vi "Download Package.vi"(7 "version (latest)":string, 8 "error in":errorcluster, 9 "download all dependencies? (T)":bool=TRUE, 10 "destination folder":path, 11 "package name":string) -> (0 "error out":errorcluster)   [LabVIEW 2014, in "NIPM_API.lvlib"]
doc: "Downloads the package and all its dependencies from registered feeds to a destination folder.\n\nINPUT(s)\n<B>Package name</B>: Specifies the package name of the package you want to download. The package must be in one of your registered feeds.\n\n<B>Destination folder</B>: Specifies the folder to place the downloaded package file(s).\n\n<B>Version (latest)</B>: Specifies the version of the package you want to download. If this input is left unwired, this VI will download the latest version of the package in your registered feeds by default.\n\n<B>Download all dependencies</B>: If you set this to TRUE, this VI will download both the specified package and all of its dependencies."
uses:
  NIPM_API.lvlib
panel:
  out "cmd standard output":string
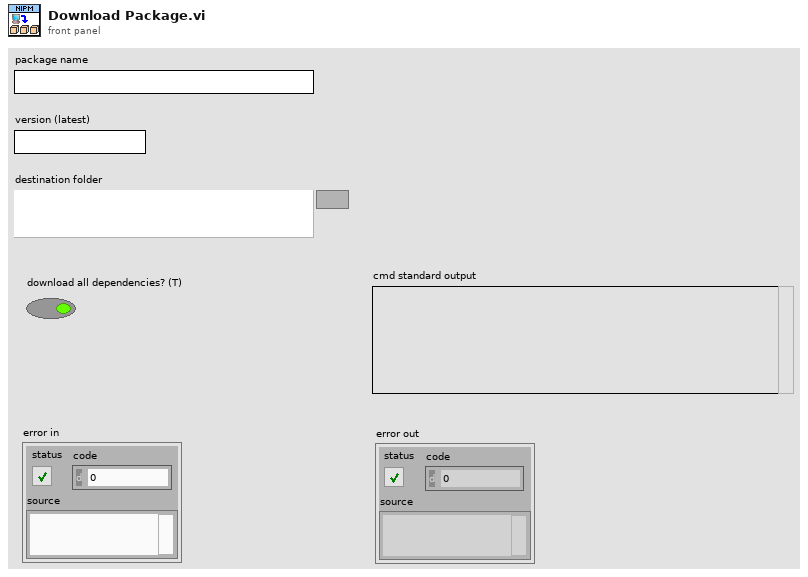
[diagram p1: front panel]
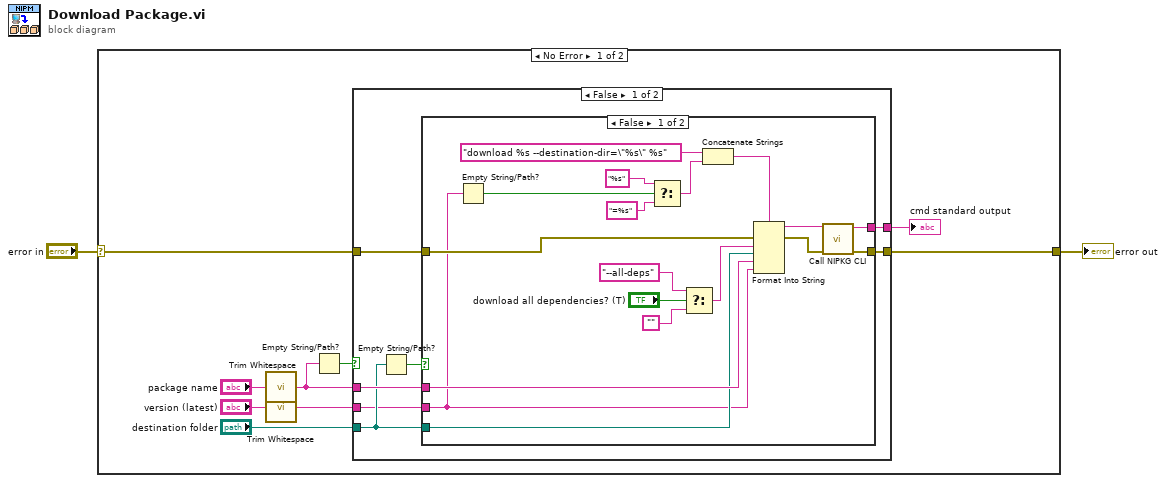
[diagram p0: block diagram]
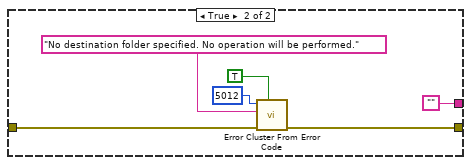
[diagram p2: hidden frame]
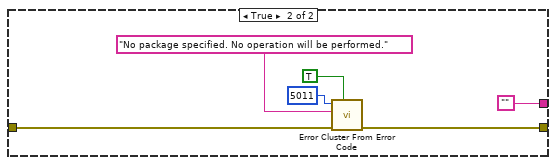
[diagram p3: hidden frame]
diagram:
  n1 = case shown="No Error" "error in" {
    selector: "error in" -> [w11 w49]
    tunnel: [w7 w49] -> w1
    frame No Error {
      n2 = call <vilib>:"Trim Whitespace.vi"("string"="package name") -> ("trimmed string"=w6:string)  [unwired: 1 in]
      n3 = call <vilib>:"Trim Whitespace.vi"("string"="version (latest)") -> ("trimmed string"=w3:string)  [unwired: 1 in]
      n4 = Empty String/Path?(string/path=w6) -> (empty?=w8:bool)
      n5 = case shown="False" w8 {
        tunnel: w11 -> [w18 w44]
        tunnel: "destination folder" -> [w14 _]
        tunnel: w6 -> [w17 _]
        tunnel: [w16 w45] -> w7
        tunnel: [w15 ""] -> w5
        tunnel: w3 -> [w12 _]
        frame False {
          n6 = Empty String/Path?(string/path=w14) -> (empty?=w13:bool)
          n7 = case shown="False" w13 {
            tunnel: w18 -> [w36 w39]
            tunnel: w17 -> [w29 _]
            tunnel: [w28 w38] -> w16
            tunnel: [w27 ""] -> w15
            tunnel: w14 -> [w26 _]
            tunnel: w12 -> [w24 _]
            frame False {
              n8 = Empty String/Path?(string/path=w24) -> (empty?=w25:bool)
              n9 = Select(t="%s", s=w25, f="=%s") -> (s? t:f=w21:string)
              n10 = Select(t="--all-deps", s="download all dependencies? (T)", f="") -> (s? t:f=w31:string)
              n11 = Concatenate Strings("download %s --destination-dir=\"%s\" %s" ("format string"), w21) -> (w20:string)
              n12 = Format Into String(format string=w20, error in=w36, w31, w26, w29, w24) -> (resulting string=w35:string, error out=w34:errorcluster)  [unwired: 1 in]
              n13 = call "Call NIPKG CLI.vi"("error in (no error)"=w34, "command"=w35) -> ("error out"=w28:errorcluster, "command line standard output"=w27:string)  [unwired: 8 in]
            }
            frame True {
              n14 = call <vilib>:"Error Cluster From Error Code.vi"("show call chain? (False)"=TRUE, "error in (no error)"=w39, "error message (\"\")"="No destination folder specified. No operation will be performed.", "error code (0)"=5012) -> ("error out"=w38:errorcluster)  [unwired: 5 in]
            }
          }
        }
        frame True {
          n15 = call <vilib>:"Error Cluster From Error Code.vi"("show call chain? (False)"=TRUE, "error in (no error)"=w44, "error message (\"\")"="No package specified. No operation will be performed.", "error code (0)"=5011) -> ("error out"=w45:errorcluster)  [unwired: 5 in]
        }
      }
      "cmd standard output" <- w5
    }
    frame Error {
    }
  }
  "error out" <- w1
